vi "Headers.vi"(8 "error in (no error)":errorcluster, 11 "LabVIEW Web Service Request":refnum<class "Web Request.lvclass">) -> (0 "error out":errorcluster, 3 "LabVIEW Web Service Request out":refnum<class "Web Request.lvclass">)   [LabVIEW 2015]
doc: "Sets all required headers by the SSE connection"
uses:
  <vilib>/wsapi/Web Request.lvclass
  Configuration/Global_Configurations.vi
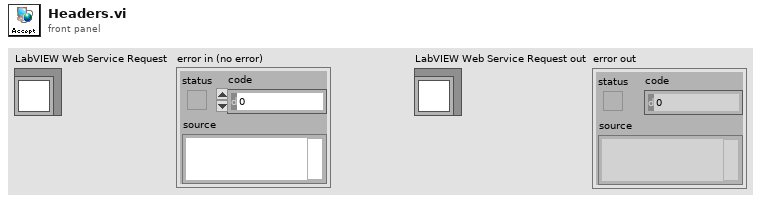
[diagram p1: front panel]
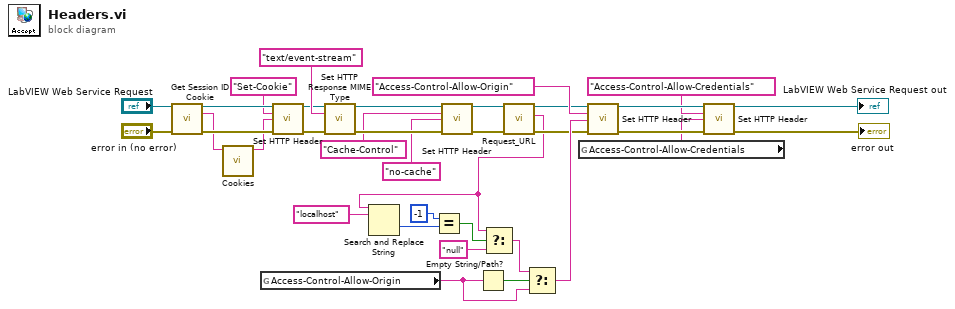
[diagram p0: block diagram]
diagram:
  n1 = call <vilib>:"Get Session ID Cookie.vi"("LabVIEW Web Service Request"="LabVIEW Web Service Request", "error in (no error)"="error in (no error)") -> ("LabVIEW Web Service Request out"=w29:refnum<class "Web Request.lvclass">, "session ID cookie"=w23:string, "error out"=w30:errorcluster)  [unwired: 11 in]
  n2 = call "Cookies.vi"("ID cookie"=w23) -> ("cookie header"=w28:string)  [unwired: 10 in]
  n3 = global read "Global_Configurations.vi" "Access-Control-Allow-Origin"() -> (w15:string)
  n4 = call <vilib>:"Set HTTP Header.vi"("LabVIEW Web Service Request"=w29, "header"="Set-Cookie", "header value"=w28, "error in (no error)"=w30) -> ("LabVIEW Web Service Request out"=w26:refnum<class "Web Request.lvclass">, "error out"=w25:errorcluster)  [unwired: 10 in]
  n5 = call <vilib>:"Set HTTP Response MIME Type.vi"("LabVIEW Web Service Request"=w26, "MIME type (text/html)"="text/event-stream" ("header"), "error in (no error)"=w25) -> ("LabVIEW Web Service Request out"=w35:refnum<class "Web Request.lvclass">, "error out"=w34:errorcluster)  [unwired: 11 in]
  n6 = call <vilib>:"Set HTTP Header.vi"("LabVIEW Web Service Request"=w35, "header"="Cache-Control", "header value"="no-cache", "error in (no error)"=w34) -> ("LabVIEW Web Service Request out"=w11:refnum<class "Web Request.lvclass">, "error out"=w10:errorcluster)  [unwired: 10 in]
  n7 = Empty String/Path?(string/path=w15) -> (empty?=w16:bool)
  n8 = call "Request_URL.vi"("error in (no error)"=w10, "LabVIEW Web Service Request"=w11) -> ("error out"=w8:errorcluster, "Request URL"=w1:string, "LabVIEW Web Service Request out"=w9:refnum<class "Web Request.lvclass">)  [unwired: 7 in]
  n9 = Search and Replace String(input string=w1, search string="localhost") -> (offset past replacement=w4:i32)  [unwired: 6 in, 3 out]
  n10 = Equal?(x=-1, y=w4) -> (x = y?=w2:bool)
  n11 = Select(t=w1, s=w2, f="null") -> (s? t:f=w7:string)
  n12 = Select(t=w7, s=w16, f=w15) -> (s? t:f=w14:string)
  n13 = global read "Global_Configurations.vi" "Access-Control-Allow-Credentials"() -> (w13:string)
  n14 = call <vilib>:"Set HTTP Header.vi"("LabVIEW Web Service Request"=w9, "header"="Access-Control-Allow-Origin", "header value"=w14, "error in (no error)"=w8) -> ("LabVIEW Web Service Request out"=w21:refnum<class "Web Request.lvclass">, "error out"=w20:errorcluster)  [unwired: 10 in]
  n15 = call <vilib>:"Set HTTP Header.vi"("LabVIEW Web Service Request"=w21, "header"="Access-Control-Allow-Credentials", "header value"=w13, "error in (no error)"=w20) -> ("LabVIEW Web Service Request out"=→"LabVIEW Web Service Request out":refnum<class "Web Request.lvclass">, "error out"=→"error out":errorcluster)  [unwired: 10 in]
